vi "EX-OR GATE.vi"() -> ()   [LabVIEW 2021]
panel:
  out "Boolean 3":bool
  in  "Boolean 2":bool
  in  "Boolean":bool
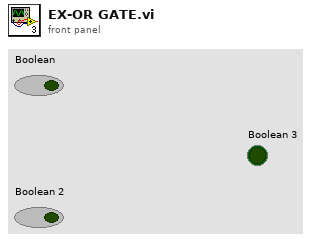
[diagram p1: front panel]
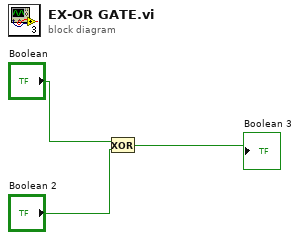
[diagram p0: block diagram]
diagram:
  n1 = Exclusive Or(1:"Boolean 2", 2:"Boolean") -> (0:→"Boolean 3":bool)
